vi "libssh2_knownhost_readline.vi"(8 "error in (no error)":errorcluster, 9 "type (OpenSSH)":T1, 10 "line":string, 11 "host key database":T2) -> (0 "error out":errorcluster)   [LabVIEW 2017, in "libssh2.lvlib"]
doc: "Read a host key from a string and add it to a host key database."
uses:
  libssh2.lvlib
  Host Key Database Refnum.ctl
  Host Key File Type.ctl
  Not A Host Key Database.vi
  <vilib>/Utility/error.llb/Error Cluster From Error Code.vi
  Global Settings.vi
  Read Host Key Database Refnum.vi
  <vilib>/Utility/semaphor.llb/Acquire Semaphore.vi
  <vilib>/Utility/semaphor.llb/Release Semaphore.vi
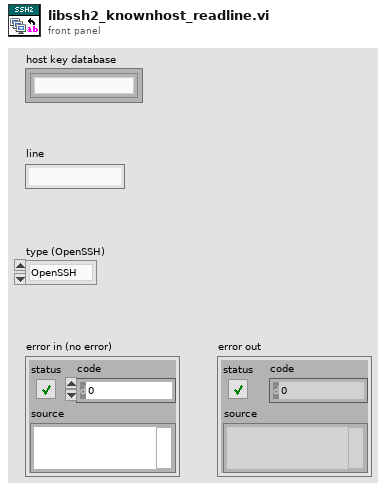
[diagram p1: front panel]
types:
  T1 = typedef "libssh2.lvlib/Host Key File Type.ctl" = enum16{"OpenSSH"}
  T2 = typedef "libssh2.lvlib/Host Key Database Refnum.ctl" = refnum<k1>
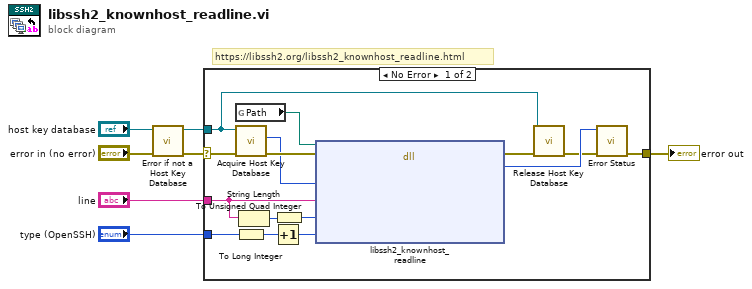
[diagram p0: block diagram]
diagram:
  # "https://libssh2.org/libssh2_knownhost_readline.html"
  n1 = call "Error if not a Host Key Database.vi"("error in (no error)"="error in (no error)", "host key database"="host key database") -> ("error out"=w3:errorcluster, "host key database out"=w1:T2)  [unwired: 8 in]
  n2 = case shown="No Error" w3 {
    selector: w3 -> [w21 w23]
    tunnel: [w20 w23] -> w7
    tunnel: "line" -> [w12 _]
    tunnel: "type (OpenSSH)" -> [w22 _]
    tunnel: w1 -> [w8 _]
    frame No Error {
      n3 = global read "Global Settings.vi" "Path"() -> (w16:path)
      n4 = call "Acquire Host Key Database.vi"("error in (no error)"=w21, "host key database"=w8) -> ("error out"=w18:errorcluster, "LIBSSH2_KNOWNHOSTS*"=w17:u64)  [unwired: 8 in]
      n5 = To Long Integer(number=w22) -> (32bit integer=w14:i32)
      n6 = String Length(string=w12) -> (length=w11:i32)
      n7 = Increment(x=w14) -> (x+1=w13:i32)
      n8 = To Unsigned Quad Integer(1:w11) -> (0:w10:u64)
      n9 = dll-call lib="?" fn="libssh2_knownhost_readline"(path in=w16, error in=w18, "hosts"=w17, "line"=w12, "len"=w10, "type"=w13) -> (error out=w19:errorcluster, "return value"=w15:i32)  [unwired: 5 in, 1 out]
      n10 = call "Release Host Key Database.vi"("error in (no error)"=w19, "host key database"=w8) -> ("error out"=w9:errorcluster)  [unwired: 9 in]
      n11 = call "Error Status.vi"("error in (no error)"=w9, "return value"=w15) -> ("error out"=w20:errorcluster)  [unwired: 8 in, 1 out]
    }
    frame Error {
    }
  }
  "error out" <- w7
